vi "Connect.vi"(8 "error in (no error)":errorcluster, 10 "Connection":T1 {"Custom Data" format="%.0x"}, 11 "CIF_Iceoryx_PCAP":refnum<class "CIF_Iceoryx_PCAP_Universal.lvclass">) -> (0 "error out":errorcluster, 3 "CIF_Iceoryx_PCAP":refnum<class "CIF_Iceoryx_PCAP_Universal.lvclass">)   [LabVIEW 2021, in "CIF_Iceoryx_PCAP_Universal.lvclass"]
uses:
  CIF_Iceoryx_PCAP_Universal.lvclass
  ChannelCommon/typedef/New FIFO Instance Response.ctl
  D:/dev/Packages/CIF_Channels_Core/src/CIFChannels/CIFChannels.lvclass
  CIFChannels/CIFChannels.lvclass/CIFChannels.ctl
  CIF_Iceoryx_PCAP_Universal.lvclass/CIF_Iceoryx_PCAP_Universal.ctl
  <vilib>/CIF Foundation/CIF Iceoryx/typedef/CIF Pcap Subscriber Configuration.ctl
  ChannelCommon/typedef/Channel State.ctl
  CIF_Iceoryx_Chan/Typedef/Iceoryx Channel Error.ctl
  Accessors/Write CIF Subscriber Refnum.vi
  CIFChannels/Accessors/Read Name.vi
  CIFChannels/Accessors/Read Direction.vi
  CIFChannels/Accessors/Read Pattern.vi
  CIFChannels/Accessors/Read FIFO Backpressure.vi
  <vilib>/CIF Foundation/CIF Iceoryx/SubVIs/Get Path.vi
  <vilib>/CIF Foundation/CIF Utilities/File/File/File Not Found Error Update.vi
  <vilib>/CIF Foundation/CIF Iceoryx/SubVIs/Convert Error.vi
  <vilib>/CIF Foundation/CIF Iceoryx/SubVIs/Add Error.vi
  <vilib>/CIF Foundation/CIF Iceoryx/Refnum/CIF Subscriber to Refnum.vi
  <vilib>/Utility/error.llb/Trim Whitespace.vi
  <vilib>/CIF Foundation/CIF Iceoryx/SubVIs/Add Error Core.vi
  <vilib>/CIF Foundation/CIF Utilities/File/SubVIs/File Not Found Error Core.vi
  <vilib>/CIF Foundation/CIF Iceoryx/SubVIs/Convert Error Core.vi
  CIF_Iceoryx_Chan/SubVIs/Iceoryx Channel Errors Core.vi
  ChannelCommon/ChannelCommon.lvlib
  CIFChannels/CIFChannels.lvclass
  CIF_Iceoryx_Chan/CIF_Iceoryx_Chn.lvclass
  <vilib>/CIF Foundation/CIF Iceoryx/Iceoryx.lvlib
  Iceorxy Utilities/Iceoryx Channel Utilities.lvlib
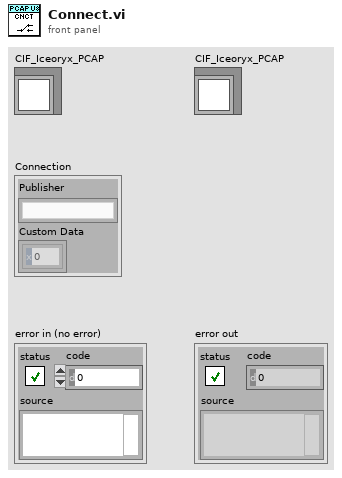
[diagram p1: front panel]
types:
  T1 = typedef "ChannelCommon.lvlib/New FIFO Instance Response.ctl" = cluster{"Publisher":string, "Custom Data":u8[]}
  T2 = typedef "Iceoryx.lvlib/CIF Pcap Subscriber Configuration.ctl" = cluster{"Name":string, "Topic":string, "Link Type":u32, "Backpressure":bool}
  T3 = typedef "ChannelCommon.lvlib/Channel State.ctl" = enum8{"Creating", "Disconnected", "Connecting", "Connected", "Destroyed"}
  T4 = typedef "CIF_Iceoryx_Chn.lvclass/Iceoryx Channel Error.ctl" = enum16{"Type Mismatch", "Name Mismatch", "Override Required"}
  T5 = typedef "ChannelCommon.lvlib/Direction.ctl" = enum8{"Publisher", "Subscriber"}
  T6 = typedef "ChannelCommon.lvlib/Channel Pattern.ctl" = enum8{"Unknown", "Tag", "FIFO", "MultiFIFO", "BackpressureFIFO"}
  T7 = typedef "CIF_Iceoryx_PCAP_Universal.lvclass/Buffer Configuration Data.ctl" = cluster{"Backpressure":bool}
  T8 = typedef "Iceoryx.lvlib/CIF Subscriber Refnum.ctl" = cluster{"refnum":u64, "CIF Sub":enum8{"cifsub"}}
  T9 = typedef "Iceoryx.lvlib/CIF Pcap Publisher Info.ctl" = cluster{"Type":string, "Link Type":u32, "Max Elements in Array":u32, "Backpressure Queue Depth":u32, "Best Effort Queue Depth":u32}
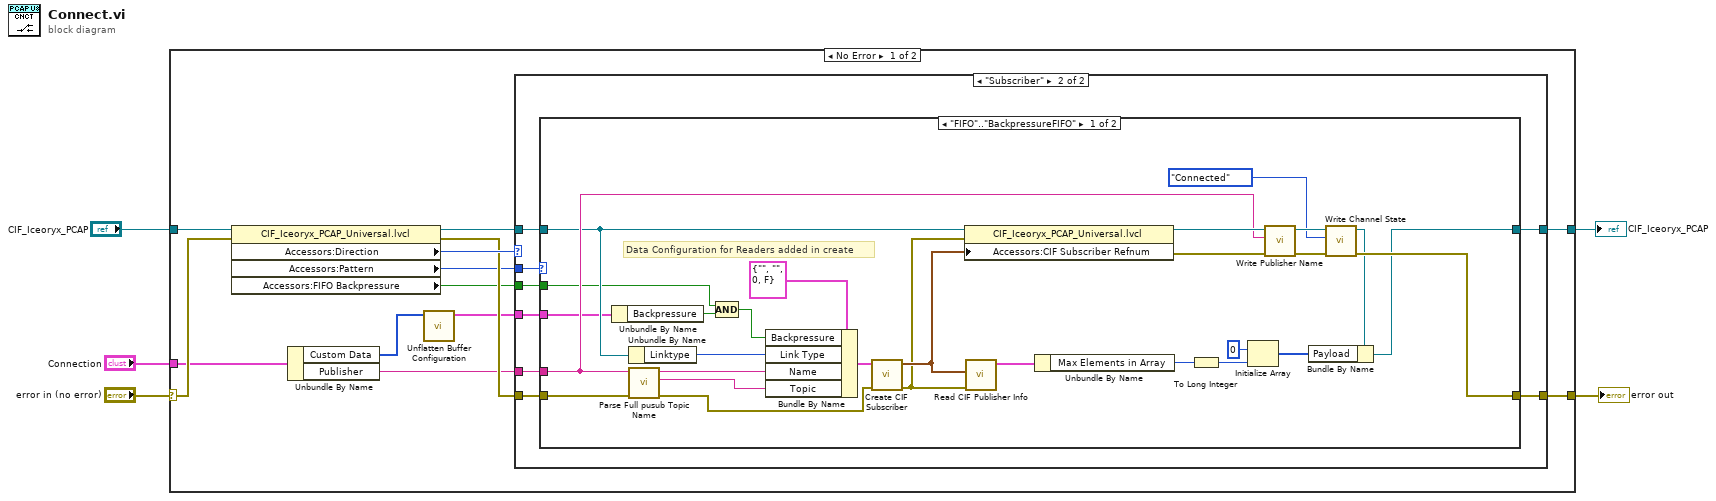
[diagram p0: block diagram]
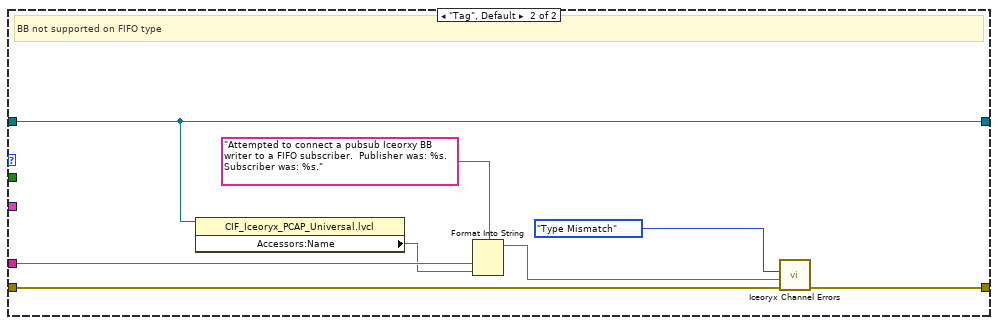
[diagram p3: hidden frame]
diagram:
  n1 = case shown="No Error" "error in (no error)" {
    selector: "error in (no error)" -> [w18 w66]
    tunnel: [w13 w66] -> w4
    tunnel: [w15 w65] -> w1
    tunnel: "CIF_Iceoryx_PCAP" -> [w9 w65]
    tunnel: "Connection" -> [w12 _]
    frame No Error {
      n2 = property class="CIF_Iceoryx_PCAP_Universal.lvcl"(reference=w9, error in=w18) -> (reference out=w17:refnum<class "CIF_Iceoryx_PCAP_Universal.lvclass">, error out=w14:errorcluster, "Accessors:Direction"=w16:T5, "Accessors:Pattern"=w10:T6, "Accessors:FIFO Backpressure"=w8:bool)
      n3 = Unbundle By Name(w12) -> ("Custom Data"=w7:u8[], "Publisher"=w11:string)
      n4 = call "Unflatten Buffer Configuration.vi"("Flattened Configuration"=w7) -> ("Buffer Configuration"=w6:T7)  [unwired: 10 in]
      n5 = case shown="\"Subscriber\"" w16 {
        tunnel: w17 -> [w20 w26]
        tunnel: [w20 w25] -> w15
        tunnel: w14 -> [w19 w28]
        tunnel: w11 -> [_ w27]
        tunnel: [w19 w24] -> w13
        tunnel: w10 -> [_ w23]
        tunnel: w8 -> [_ w22]
        tunnel: w6 -> [_ w21]
        frame "Publisher" {
          # "No connection step needed for publishers"
        }
        frame "Subscriber" {
          n6 = case shown="\"FIFO\"..\"BackpressureFIFO\"" w23 {
            tunnel: w28 -> [w40 w63]
            tunnel: w27 -> [w41 w61]
            tunnel: w26 -> [w37 w59]
            tunnel: [w42 w59] -> w25
            tunnel: [w56 w62] -> w24
            tunnel: w22 -> [w30 _]
            tunnel: w21 -> [w32 _]
            frame "FIFO".."BackpressureFIFO" {
              # "Data Configuration for Readers added in create"
              n7 = Unbundle By Name(w32) -> ("Backpressure"=w31:bool)
              n8 = Unbundle By Name(w37) -> ("Linktype"=w36:u32)
              n9 = call "Parse Full pusub Topic Name.vi"("error in"=w40, "Full pubsub Topic Name"=w41) -> ("error out"=w33:errorcluster, "Topic"=w34:string, "Plugin name"=w35:string)  [unwired: 7 in]
              n10 = Compound Arithmetic op=AND(w30, w31) -> (w29:bool)
              n11 = Bundle By Name(cluster=T2 {"Name"="", "Topic"="", "Link Type"=0, "Backpressure"=FALSE} ("CIF Pcap Subscriber Configuration"), "Backpressure"=w29, "Link Type"=w36, "Name"=w35, "Topic"=w34) -> (w38:T2)
              n12 = call <vilib>:"Create CIF Subscriber.vi"("error in (no error)"=w33, "CIF Pcap Subscriber Configuration"=w38) -> ("error out"=w51:errorcluster, "CIF Subscriber Refnum"=w52:T8)  [unwired: 8 in]
              n13 = property class="CIF_Iceoryx_PCAP_Universal.lvcl"(reference=w37, error in=w51, "Accessors:CIF Subscriber Refnum"=w52) -> (reference out=w45:refnum<class "CIF_Iceoryx_PCAP_Universal.lvclass">, error out=w44:errorcluster)
              n14 = call <vilib>:"Read CIF Publisher Info.vi"("error in (no error)"=w51, "CIF Subscriber Refnum"=w52) -> ("CIF Publisher Info"=w46:T9)  [unwired: 8 in, 1 out]
              n15 = Unbundle By Name(w46) -> ("Max Elements in Array"=w50:u32)
              n16 = To Long Integer(number=w50) -> (32bit integer=w47:i32)
              n17 = Initialize Array(u8 0 ("Numeric"), w47) -> (w49:u8[])
              n18 = call "Write Publisher Name.vi"("error in (no error)"=w44, "Publisher Name"=w41, "CIFChannels in"=w45) -> ("error out"=w54:errorcluster, "CIFChannels out"=w55:refnum<class "CIF_Iceoryx_PCAP_Universal.lvclass">)  [unwired: 7 in]
              n19 = call "Write Channel State.vi"("error in (no error)"=w54, "Channel State"=Channel_State."Connected", "CIFChannels in"=w55) -> ("error out"=w56:errorcluster, "CIFChannels out"=w43:refnum<class "CIF_Iceoryx_PCAP_Universal.lvclass">)  [unwired: 7 in]
              n20 = Bundle By Name(cluster=w43, "Payload"=w49) -> (w42:refnum<class "CIF_Iceoryx_PCAP_Universal.lvclass">)
            }
            frame "Tag", Default {
              # "BB not supported on FIFO type"
              n21 = property class="CIF_Iceoryx_PCAP_Universal.lvcl"(reference=w59) -> ("Accessors:Name"=w57:string)  [unwired: 1 in, 2 out]
              n22 = Format Into String(format string="Attempted to connect a pubsub Iceorxy BB writer to a FIFO subscriber.  Publisher was: %s. Subscriber was: %s." ("String to Append"), w61, w57) -> (resulting string=w60:string)  [unwired: 2 in, 1 out]
              n23 = call "Iceoryx Channel Errors.vi"("error in (no error)"=w63, "String to Append"=w60, "Error"=Iceoryx_Channel_Error."Type Mismatch") -> ("error out"=w62:errorcluster)  [unwired: 8 in]
            }
          }
        }
      }
    }
    frame Error {
    }
  }
  "error out" <- w4
  "CIF_Iceoryx_PCAP" <- w1
